vi "Get Device Parameters.vi"(8 "error in":errorcluster, 11 "custom device ref":T2=18446744073709551615 format="%.0x") -> (0 "error out":errorcluster, 2 "device parameters":T1 {"coupling mode" items=["API429_CHANNEL_COUPLING_EXT", "API429_CHANNEL_COUPLING_DUAL", "API429_CHANNEL_COUPLING_INT"]}, 3 "custom device ref out":T2 format="%.0x")   [LabVIEW 2020, in "AIM ARINC 429 Scripting.lvlib"]
doc: "Returns AIM hardware device parameters such as <b>pxi slot</b>."
uses:
  AIM ARINC 429 Scripting.lvlib
  <vilib>/NI VeriStand/Custom Device API/Custom Device API.lvlib
  Shared/Device Parameters.ctl
  Constants.vi
  <vilib>/NI VeriStand/Custom Device API/Get Item Property (I32).vi
  <vilib>/NI VeriStand/Custom Device API/Custom Device Item Ref.ctl
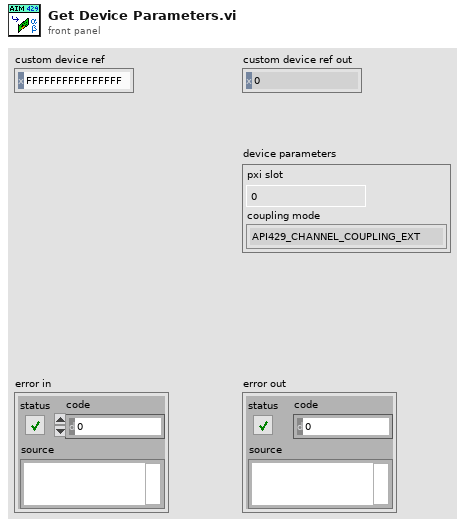
[diagram p1: front panel]
types:
  T1 = typedef "Device Parameters.ctl" = cluster{"pxi slot":u8, "coupling mode":u32}
  T2 = typedef "Custom Device API.lvlib/Custom Device Item Ref.ctl" = u64
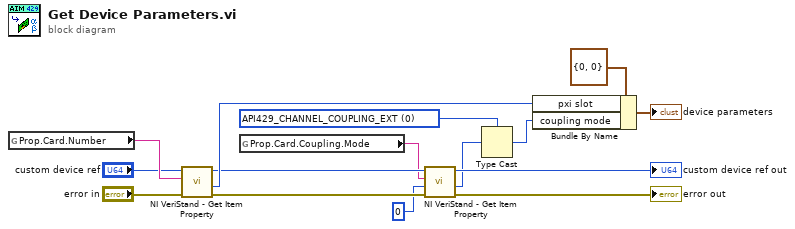
[diagram p0: block diagram]
diagram:
  w2 = u32 0 items=["API429_CHANNEL_COUPLING_EXT", "API429_CHANNEL_COUPLING_DUAL", "API429_CHANNEL_COUPLING_INT"] ("coupling mode")
  n1 = global read "Constants.vi" "Prop.Card.Number"() -> (w14:string)
  n2 = call-poly <vilib>:"NI VeriStand - Get Item Property.vi"("error in (no error)"="error in", "Property Name"=w14, "Item Ref in"="custom device ref") -> ("error out"=w9:errorcluster, "Value"=w13:i32, "Item Ref out"=w8:T2)  [unwired: 5 in, 1 out]
  n3 = global read "Constants.vi" "Prop.Card.Coupling.Mode"() -> (w5:string)
  n4 = call-poly <vilib>:"NI VeriStand - Get Item Property.vi"("error in (no error)"=w9, "Default Value"=0, "Property Name"=w5, "Item Ref in"=w8) -> ("error out"=→"error out":errorcluster, "Value"=w3:i32, "Item Ref out"=→"custom device ref out":T2)  [unwired: 4 in, 1 out]
  n5 = Type Cast(type=w2, x=w3) -> (*(type *) &x=w1:u32)
  n6 = Bundle By Name(cluster=T1 {"pxi slot"=0, "coupling mode"=0} ("device parameters"), "pxi slot"=w13, "coupling mode"=w1) -> (→"device parameters":T1)
